vi "Subcool and Super heat.vi"(7 "LLT":dbl, 8 "SLT":dbl, 9 "SLP":dbl, 10 "Refrigerant":enum16{"R407c", "R410a", "R134a", "R22", ""}(ring), 11 "LLP":dbl) -> (0 "SupperHeat 2":dbl format="%#_4g", 1 "Evaporating Temp":dbl, 2 "Sub-Cooling":dbl format="%#_4g", 3 "Condensing Temp":dbl, 4 "Enth_Vap":dbl, 5 "Enth_Liq":dbl)   [LabVIEW 2025]
panel:
  out "Temp  DEW POINT/Vap":dbl[](array[numeric])
  out "appended path":path
  out "Temp  BUBBLE POINT/Liq":dbl[](array[numeric])
  out "Pressure":dbl[](array[numeric])
  # "111"
  # "113.1"
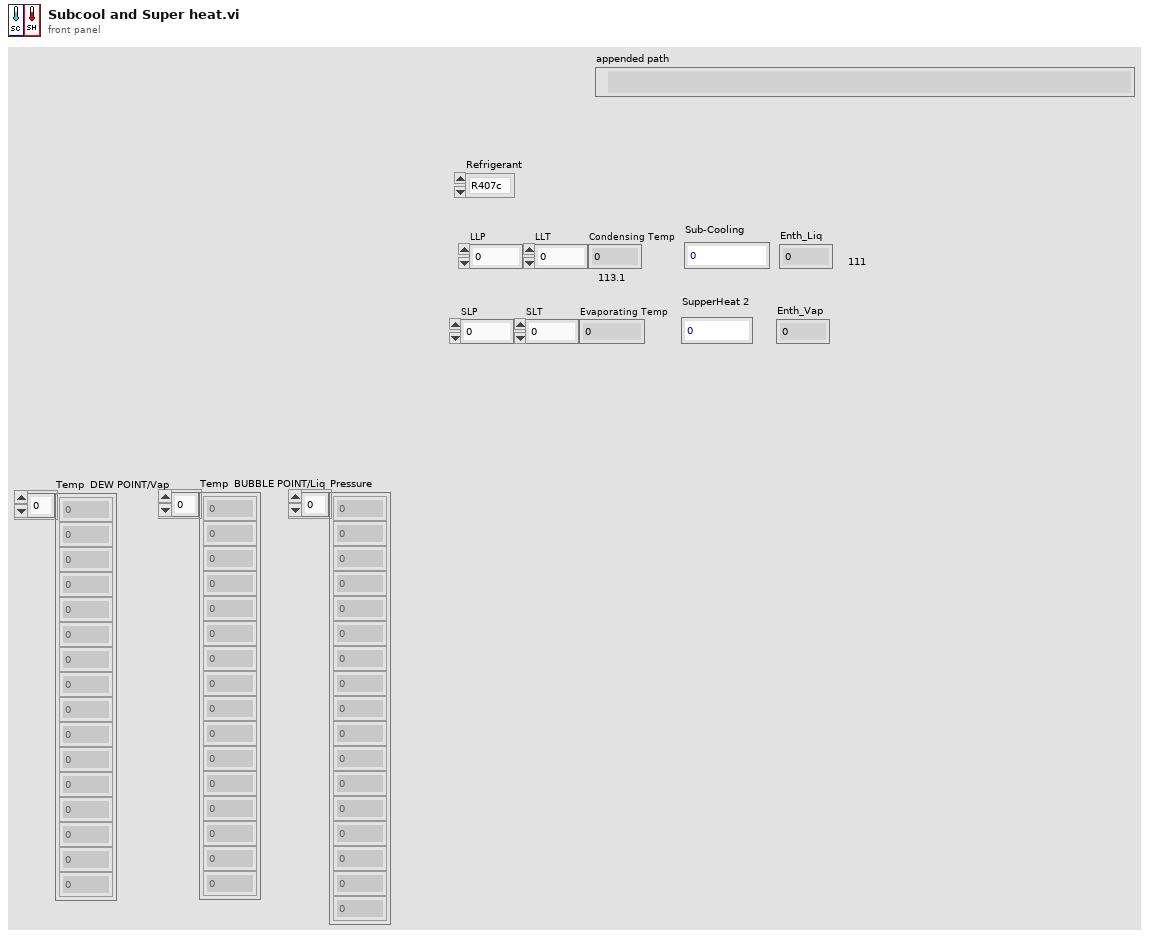
[diagram p1: front panel]
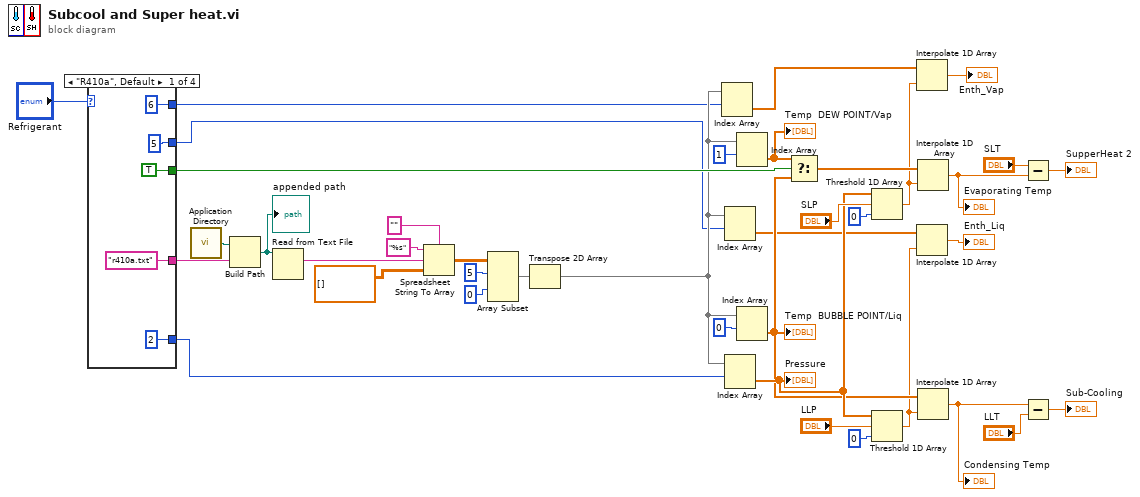
[diagram p0: block diagram]
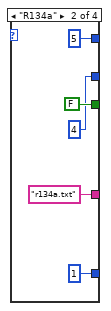
[diagram p2: hidden frame]
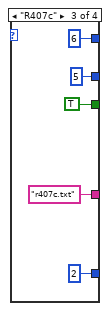
[diagram p3: hidden frame]
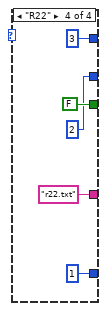
[diagram p4: hidden frame]
diagram:
  n1 = case shown="\"R410a\", Default" "Refrigerant" {
    tunnel: ["r410a.txt" ("name or relative path") "r134a.txt" ("name or relative path") "r407c.txt" ("name or relative path") "r22.txt" ("name or relative path")] -> w31
    tunnel: [2 ("index") 1 ("index") 2 ("index") 1 ("index")] -> w18
    tunnel: [TRUE FALSE TRUE FALSE] -> w14
    tunnel: [5 ("index (row)") 4 ("index (row)") 5 ("index") 2 ("index")] -> w2
    tunnel: [6 ("index (row)") 5 ("index (row)") 6 ("index") 3 ("index")] -> w1
    frame "R410a", Default {
    }
    frame "R134a" {
    }
    frame "R407c" {
    }
    frame "R22" {
    }
  }
  n2 = call <vilib>:"Application Directory.vi"() -> ("Application Directory"=w32:path)
  n3 = Build Path(base path=w32, name or relative path=w31) -> (appended path=w30:path)
  "appended path" <- w30
  n4 = Read from Text File(file (use dialog)=w30) -> (text=w33:string)  [unwired: 3 in, 3 out]
  n5 = Spreadsheet String To Array(delimiter (Tab)="", format string="%s", spreadsheet string=w33, array type (2D Dbl)=dbl[][] []) -> (array=w39:dbl[][])
  n6 = Array Subset(array=w39, index (row)=5 ("index"), index (col)=0 ("index")) -> (w20:dbl[][])  [unwired: 2 in]
  n7 = Transpose 2D Array(2D array=w20) -> (transposed array=w6:dbl[][])
  n8 = Index Array(array=w6, index (row)=w1) -> (element=w4:dbl[])  [unwired: 1 in]
  n9 = Index Array(array=w6, index (row)=w2) -> (element=w7:dbl[])  [unwired: 1 in]
  n10 = Index Array(array=w6, index (row)=w18) -> (element=w19:dbl[])  [unwired: 1 in]
  "Pressure" <- w19
  n11 = Index Array(array=w6, index (row)=1) -> (element=w13:dbl[])  [unwired: 1 in]
  "Temp  DEW POINT/Vap" <- w13
  n12 = Index Array(array=w6, index (row)=0) -> (element=w15:dbl[])  [unwired: 1 in]
  "Temp  BUBBLE POINT/Liq" <- w15
  n13 = Select(t=w13, s=w14, f=w15) -> (s? t:f=w16:dbl[])
  n14 = Threshold 1D Array(1:0 ("start index (0)"), 2:"SLP", 3:w19) -> (0:w3:dbl)
  n15 = Threshold 1D Array(1:0 ("start index (0)"), 2:"LLP", 3:w19) -> (0:w9:dbl)
  n16 = Interpolate 1D Array(1:w3, 2:w4) -> (0:→"Enth_Vap":dbl)
  n17 = Interpolate 1D Array(1:w9, 2:w7) -> (0:→"Enth_Liq":dbl)
  n18 = Interpolate 1D Array(1:w3, 2:w16) -> (0:w10:dbl)
  "Evaporating Temp" <- w10
  n19 = Interpolate 1D Array(1:w9, 2:w15) -> (0:w11:dbl)
  "Condensing Temp" <- w11
  n20 = Subtract(x="SLT", y=w10) -> (x-y=→"SupperHeat 2":dbl)
  n21 = Subtract(x=w11, y="LLT") -> (x-y=→"Sub-Cooling":dbl)
